vi "Initialize.vi"(2 "XRef":refnum<vi>) -> (1 "State Out":T1)   [LabVIEW 2012, in "IsA.xnode"]
uses:
  IsA.xnode
  State.ctl
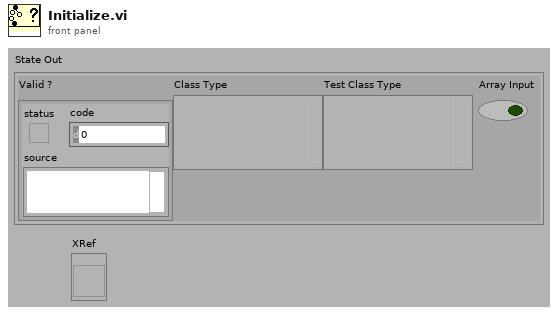
[diagram p1: front panel]
types:
  T1 = typedef "IsA.xnode/State.ctl" = cluster{"Valid ?":errorcluster, "Class Type":variant, "Test Class Type":variant, "Array Input":bool}
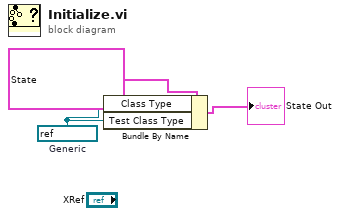
[diagram p0: block diagram]
diagram:
  w1 = refnum<vi> refnum  # Generic
  n1 = Bundle By Name(cluster=T1 {"Valid ?"={"status"=TRUE, "code"=-1, "source"="Initialised"}, "Class Type"=variant, "Test Class Type"=variant, "Array Input"=FALSE} ("State Out"), "Class Type"=w1, "Test Class Type"=w1) -> (→"State Out":T1)
